vi "Register Extract.vi"(11 "All MCS Registers":cluster{"all rows":string[][]}[](array[cluster])) -> (3 "Registers":string[][](array[string]))   [LabVIEW 2025]
panel:
  out "Numeric":i32
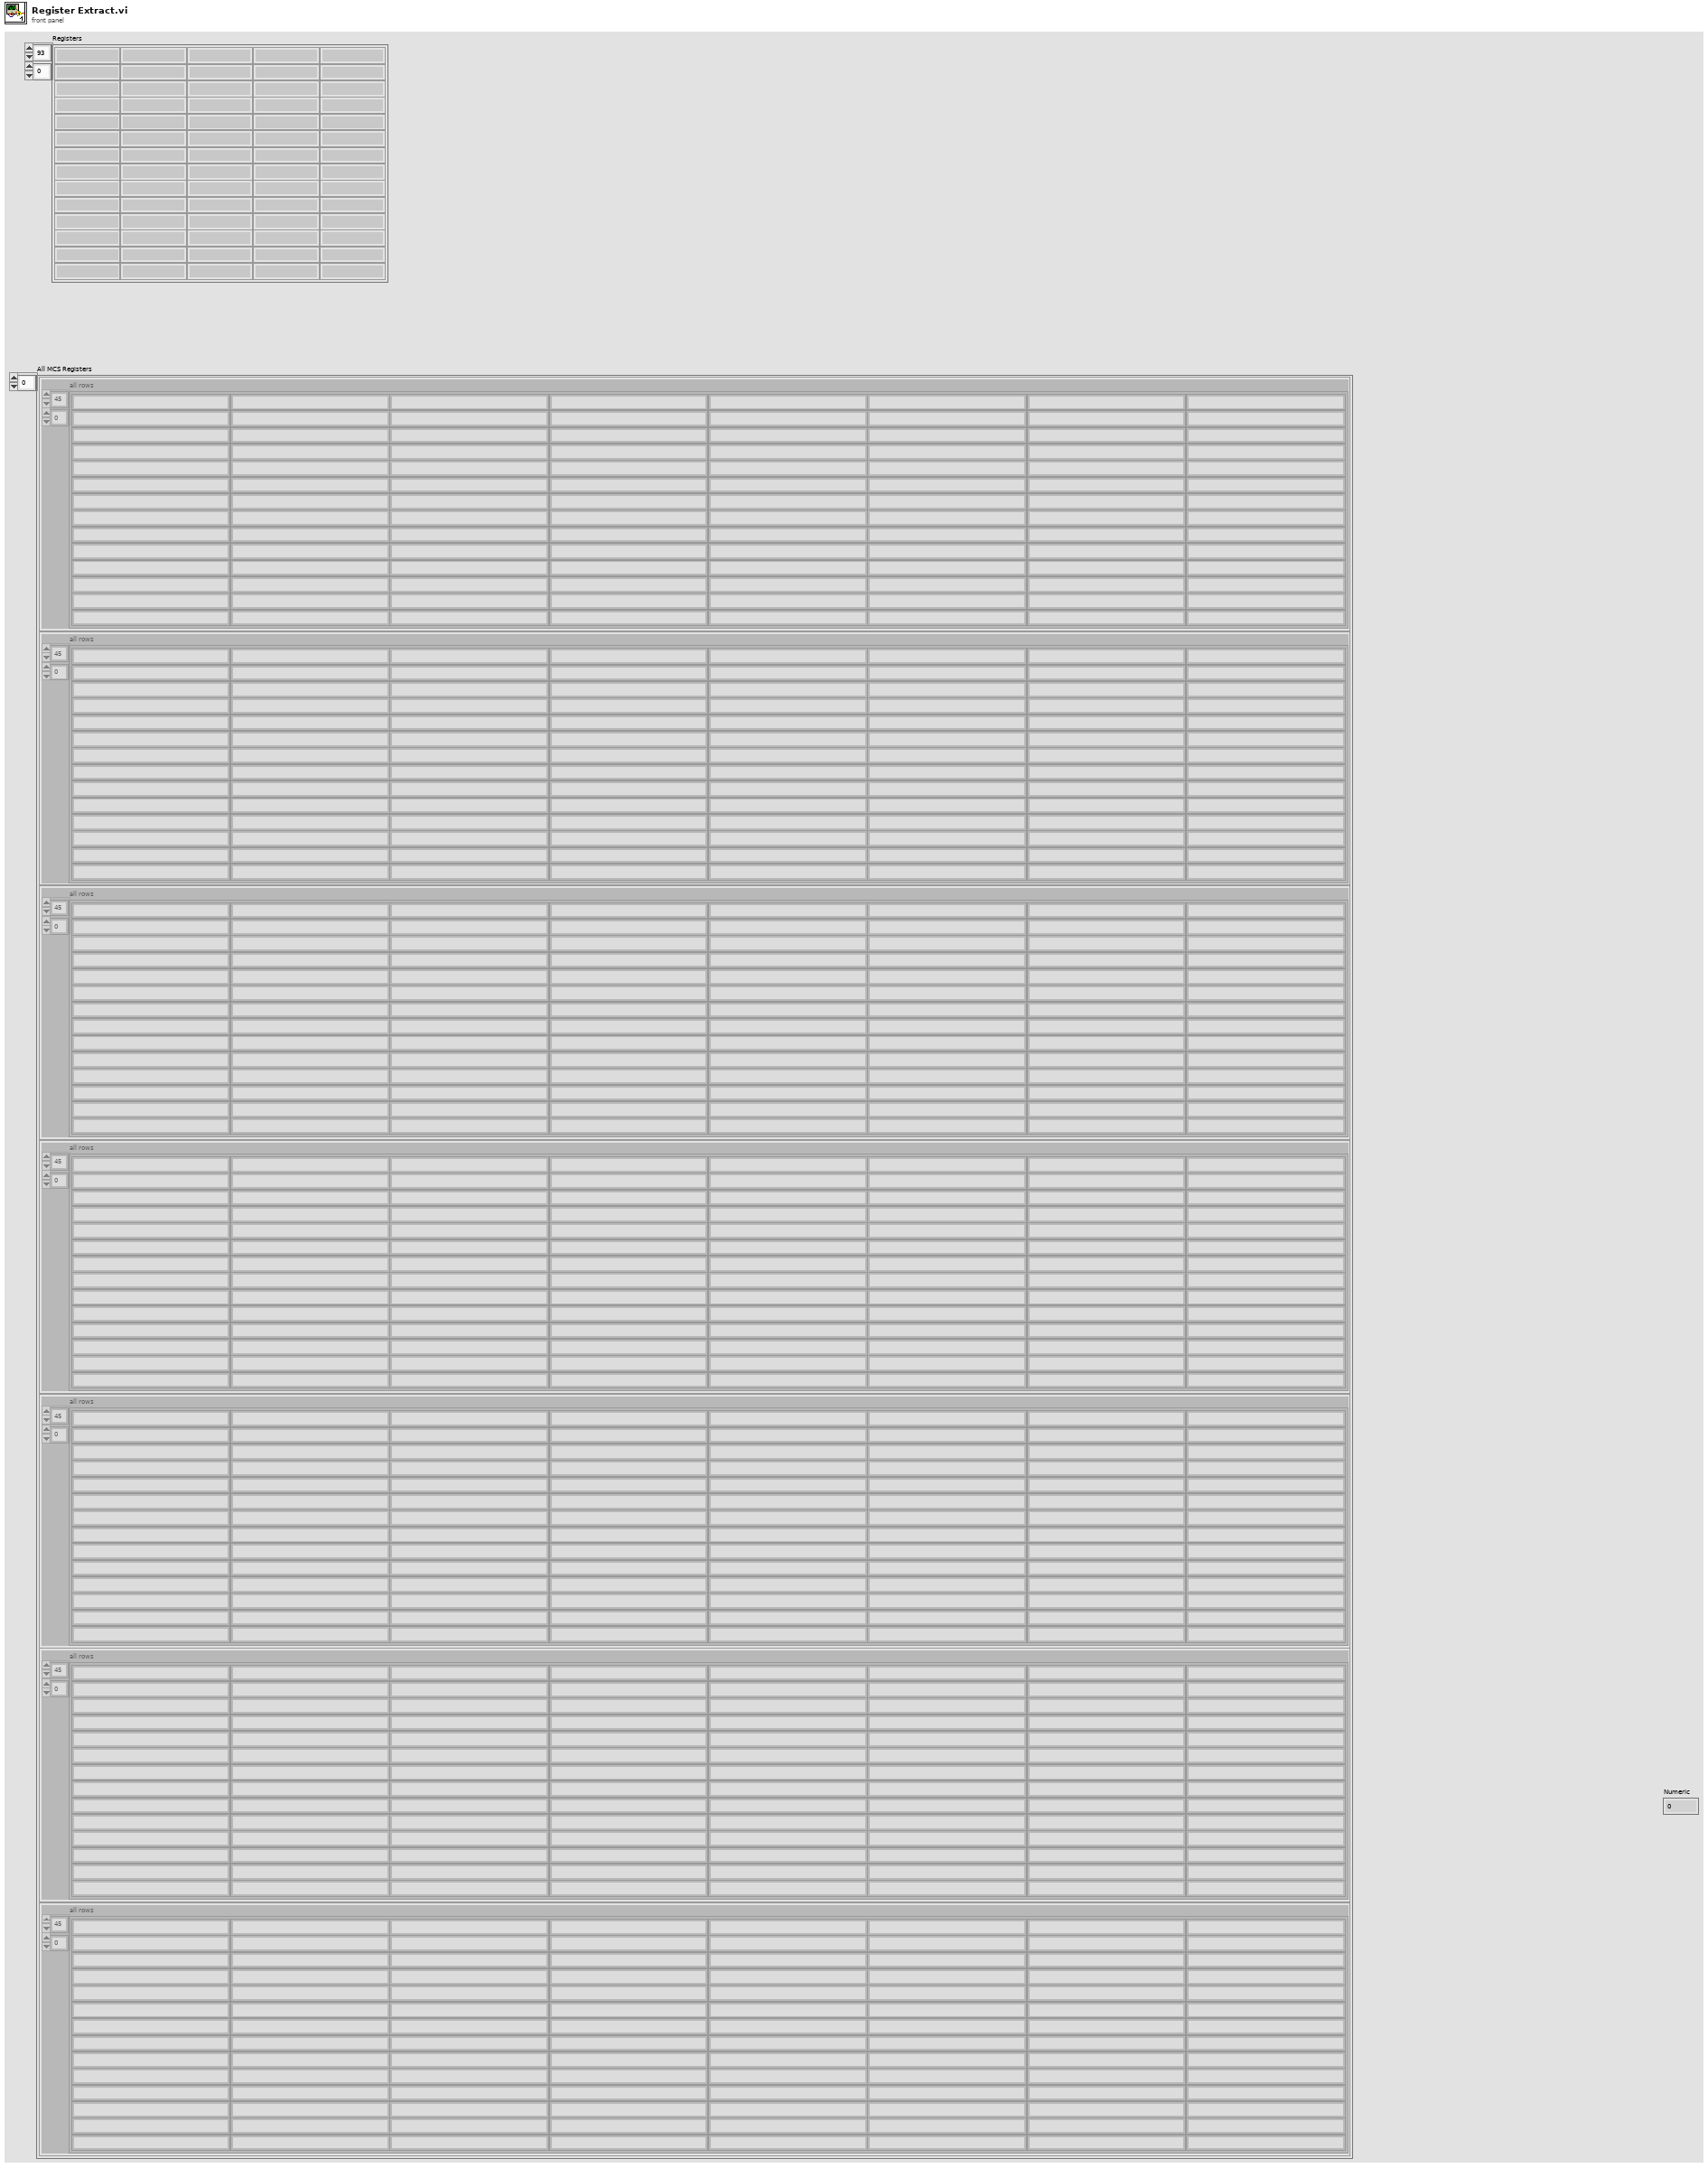
[diagram p1: front panel]
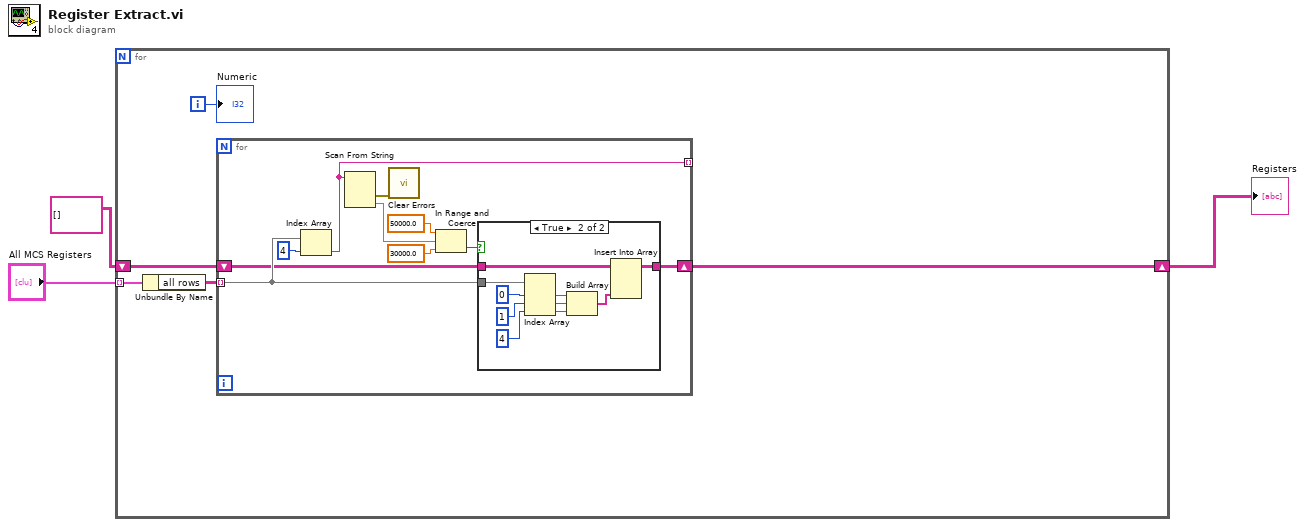
[diagram p0: block diagram]
diagram:
  n1 = for {
    tunnel: "All MCS Registers" -> [w8] mode=indexing
    shift-right: [w4] -> w1
    shift-left: string[][] [] -> [w5]
    i -> [w7]
    n2 = Unbundle By Name(w8) -> ("all rows"=w6:string[][])
    n3 = for {
      tunnel: w6 -> [w13] mode=indexing
      tunnel: [w9] -> _ mode=indexing
      shift-right: [w11] -> w4
      shift-left: w5 -> [w12]
      n4 = Index Array(array=w13, index=4) -> (element=w9:string)
      n5 = Scan From String(input string=w9) -> (error out=w18:errorcluster, output 1=w17:dbl)  [unwired: 4 in, 2 out]
      n6 = call <vilib>:"Clear Errors.vi"("error in (no error)"=w18) -> ()  [unwired: 5 in, 2 out]
      n7 = In Range and Coerce(upper limit=50000.0 ("x"), x=w17, lower limit=30000.0 ("x")) -> (In Range?=w14:bool)  [unwired: 1 out]
      n8 = case shown="True" w14 {
        tunnel: w13 -> [_ w29]
        tunnel: w12 -> [w19 w22]
        tunnel: [w19 w21] -> w11
        frame False {
        }
        frame True {
          n9 = Index Array(array=w29, index #1=0 ("index"), index #2=1 ("index"), index #3=4 ("index")) -> (element #1=w25:string, element #2=w24:string, element #3=w23:string)
          n10 = Build Array(w25, w24, w23) -> (w20:string[])
          n11 = Insert Into Array(array=w22, new element=w20) -> (w21:string[][])  [unwired: 2 in]
        }
      }
    }
    "Numeric" <- w7
  }
  "Registers" <- w1
